vi "Test Save Edited Entry.vi"(8 "error in":errorcluster, 10 "Work Folder":path, 11 "Test Data Folder":path) -> (0 "error out":errorcluster, 2 "Report":string, 3 "Passed":bool)   [LabVIEW 2026]
doc: "Tests Save Edited Entry.vi on a copy of the schema-v2 sample data. The entries of 2025-10-06 are read with Load Day.vi. The first is moved to 2025-09-20 (another UTC month); the second only gets a new description. Checks: the moved entry is gone from 2025-10.ini; it is in 2025-09.ini with its new Start Time; the other 2025-10 entry is kept; an edit within the month overwrites the row in place.\n\nInputs: Test Data Folder; Work Folder; error in. Outputs: Passed; Report; error out.\n\nGenerated by: Claude"
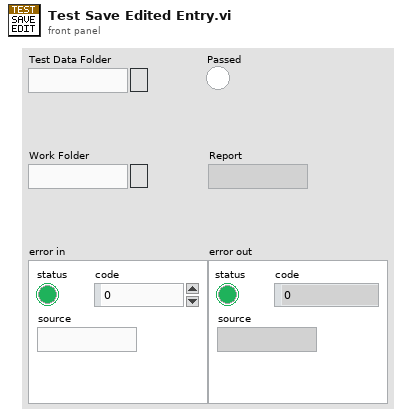
[diagram p1: front panel]
types:
  T1 = typedef "Time Entry List.ctl" = T2[]
  T2 = typedef "Time Entry.ctl" = cluster{"ID":string, "Project ID":string, "Task ID":string, "Start Time":timestamp, "End Time":timestamp, "Description":string}
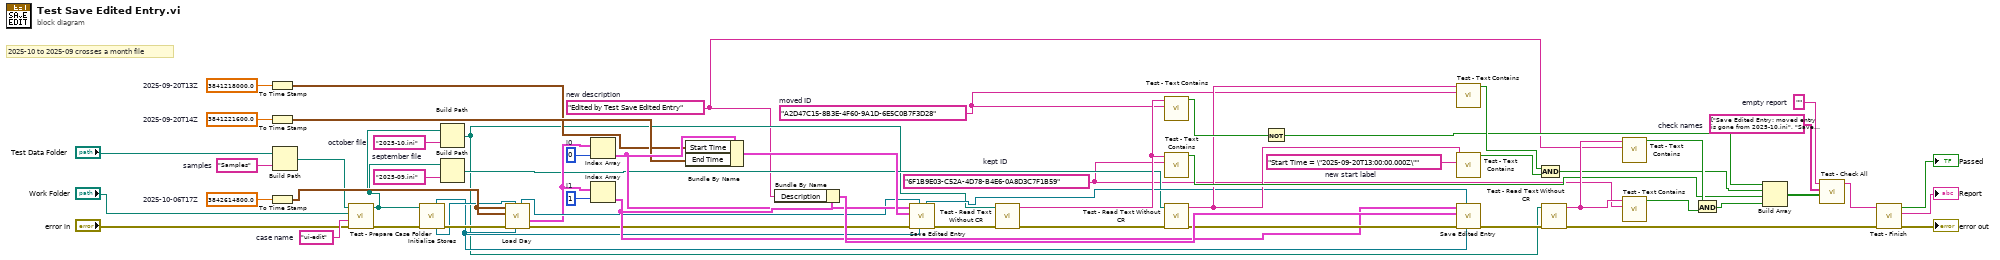
[diagram p0: block diagram]
diagram:
  w21 = string[] ["Save Edited Entry: moved entry is gone from 2025-10.ini", "Save Edited Entry: moved entry is in 2025-09.ini with its new Start Time", "Save Edited Entry: the other 2025-10 entry is kept", "Save Edited Entry: an edit within the month overwrites the row in place"]  # check names
  w20 = "Edited by Test Save Edited Entry"  # new description
  w19 = "Start Time = \"2025-09-20T13:00:00.000Z\""  # new start label
  w18 = "6F1B9E03-C52A-4D78-B4E6-0A8D3C7F1B59"  # kept ID
  w17 = "A2D47C15-8B3E-4F60-9A1D-6E5C0B7F3D28"  # moved ID
  w16 = 1  # i1
  w15 = 0  # i0
  w14 = 3841221600.0  # 2025-09-20T14Z
  w13 = 3841218000.0  # 2025-09-20T13Z
  w12 = 3842614800.0  # 2025-10-06T17Z
  w11 = "2025-09.ini"  # september file
  w10 = "2025-10.ini"  # october file
  w9 = ""  # empty report
  w8 = "ui-edit"  # case name
  w7 = "Samples"  # samples
  # "2025-10 to 2025-09 crosses a month file"
  n1 = To Time Stamp(1:w13) -> (0:w31:timestamp)
  n2 = To Time Stamp(1:w14) -> (0:w32:timestamp)
  n3 = To Time Stamp(1:w12) -> (0:w30:timestamp)
  n4 = Build Path(base path="Test Data Folder", name or relative path=w7) -> (appended path=w22:path)
  n5 = call "Test - Prepare Case Folder.vi"("error in (no error)"="error in", "Case Name"=w8, "Work Folder"="Work Folder", "Source Folder"=w22) -> ("error out"=w24:errorcluster, "Case Folder"=w23:path)  [unwired: 6 in]
  n6 = call "Initialize Stores.vi"("error in"=w24, "Data Folder"=w23) -> ("error out"=w29:errorcluster, "Time Entry Store out"=w28:refnum<class "Time Entry Store.lvclass">, "Project Store out"=w27:refnum<class "Project Store.lvclass">)  [unwired: 5 in, 2 out]
  n7 = Build Path(base path=w23, name or relative path=w10) -> (appended path=w25:path)
  n8 = Build Path(base path=w23, name or relative path=w11) -> (appended path=w26:path)
  n9 = call "Load Day.vi"("Project Store in"=w27, "Time Entry Store in"=w28, "error in"=w29, "Now"=w30, "Day"=w30) -> ("error out"=w35:errorcluster, "Day Entries"=w33:T1, "Time Entry Store out"=w34:refnum<class "Time Entry Store.lvclass">)  [unwired: 1 in, 3 out]
  n10 = Index Array(array=w33, index=w15) -> (element=w36:T2)
  n11 = Index Array(array=w33, index=w16) -> (element=w37:T2)
  n12 = Bundle By Name(cluster=w36, "Start Time"=w31, "End Time"=w32) -> (w38:T2)
  n13 = Bundle By Name(cluster=w37, "Description"=w20) -> (w51:T2)
  n14 = call "Save Edited Entry.vi"("Project Store in"=w27, "Time Entry Store in"=w34, "error in"=w35, "Edited Entry"=w38, "Original Entry"=w36) -> ("error out"=w40:errorcluster, "Time Entry Store out"=w39:refnum<class "Time Entry Store.lvclass">)  [unwired: 4 in, 1 out]
  n15 = call "Test - Read Text Without CR.vi"("error in (no error)"=w40, "File"=w25) -> ("error out"=w42:errorcluster, "Text"=w41:string)  [unwired: 8 in]
  n16 = call "Test - Text Contains.vi"("Search Text"=w17, "Text"=w41) -> ("Contains?"=w45:bool)  [unwired: 8 in, 1 out]
  n17 = call "Test - Text Contains.vi"("Search Text"=w18, "Text"=w41) -> ("Contains?"=w50:bool)  [unwired: 8 in, 1 out]
  n18 = call "Test - Read Text Without CR.vi"("error in (no error)"=w42, "File"=w26) -> ("error out"=w44:errorcluster, "Text"=w43:string)  [unwired: 8 in]
  n19 = Not(x=w45) -> (.not. x?=w46:bool)
  n20 = call "Test - Text Contains.vi"("Search Text"=w17, "Text"=w43) -> ("Contains?"=w47:bool)  [unwired: 8 in, 1 out]
  n21 = call "Test - Text Contains.vi"("Search Text"=w19, "Text"=w43) -> ("Contains?"=w48:bool)  [unwired: 8 in, 1 out]
  n22 = call "Save Edited Entry.vi"("Project Store in"=w27, "Time Entry Store in"=w39, "error in"=w44, "Edited Entry"=w51, "Original Entry"=w37) -> ("error out"=w52:errorcluster)  [unwired: 4 in, 2 out]
  n23 = And(x=w47, y=w48) -> (x .and. y?=w49:bool)
  n24 = call "Test - Read Text Without CR.vi"("error in (no error)"=w52, "File"=w25) -> ("error out"=w54:errorcluster, "Text"=w53:string)  [unwired: 8 in]
  n25 = call "Test - Text Contains.vi"("Search Text"=w20, "Text"=w53) -> ("Contains?"=w55:bool)  [unwired: 8 in, 1 out]
  n26 = call "Test - Text Contains.vi"("Search Text"=w18, "Text"=w53) -> ("Contains?"=w56:bool)  [unwired: 8 in, 1 out]
  n27 = And(x=w55, y=w56) -> (x .and. y?=w57:bool)
  n28 = Build Array(w46, w49, w50, w57) -> (w58:bool[])
  n29 = call "Test - Check All.vi"("Conditions"=w58, "Check Names"=w21, "Report in"=w9) -> ("Report out"=w59:string)  [unwired: 7 in, 1 out]
  n30 = call "Test - Finish.vi"("error in (no error)"=w54, "Report"=w59) -> ("error out"=→"error out":errorcluster, "Report out"=→"Report":string, "Passed"=→"Passed":bool)  [unwired: 7 in]
